vi "Schema.vi"(8 "error in (no error)":errorcluster, 11 "SQLite Connection In":refnum<class "Connection.lvclass">) -> (0 "error out":errorcluster, 1 "Table Names":string[](array[string]), 2 "Schema":T1, 3 "SQLite Connection Out":refnum<class "Connection.lvclass">)   [LabVIEW 2024, in "DBMigrations.lvlib"]
doc: "Get database schema: table names, column names, and column properties"
uses:
  DBMigrations.lvlib
  <vilib>/drjdpowell/SQLite Library/SQL Connection/Connection.lvclass
  Schema.ctl
  <vilib>/drjdpowell/SQLite Library/SQL Connection/Execute SQL (1D String).vi
  <vilib>/drjdpowell/SQLite Library/SQL Connection/Execute SQL.vi
  <vilib>/drjdpowell/SQLite Library/SQLite.lvlib
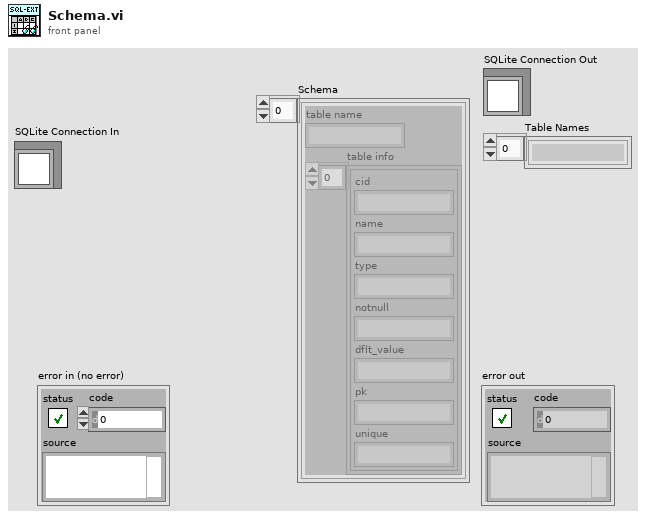
[diagram p1: front panel]
types:
  T1 = typedef "DBMigrations.lvlib/Schema.ctl" = cluster{"table name":string, "table info":cluster{"cid":string, "name":string, "type":string, "notnull":string, "dflt_value":string, "pk":string, "unique":string}[]}[]
  T2 = cluster{"table name":string, "table info":cluster{"cid":string, "name":string, "type":string, "notnull":string, "dflt_value":string, "pk":string, "unique":string}[]}
  T3 = cluster{"cid":string, "name":string, "type":string, "notnull":string, "dflt_value":string, "pk":string, "unique":string}
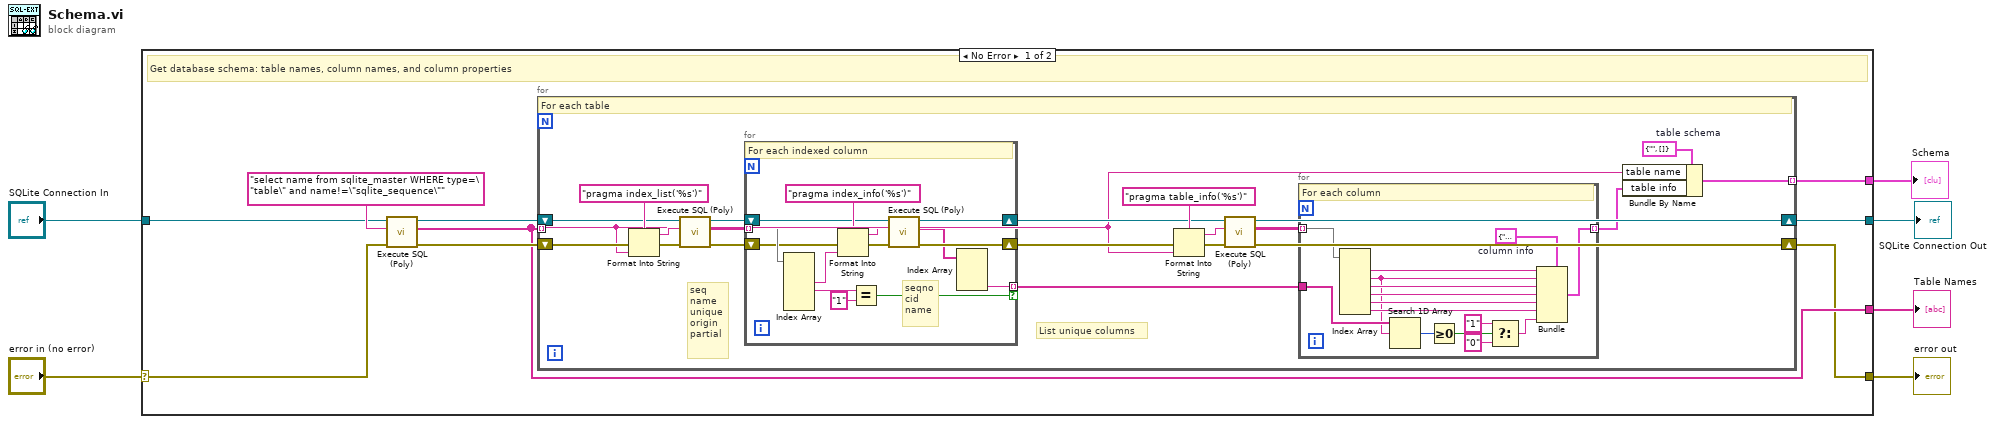
[diagram p0: block diagram]
diagram:
  n1 = case shown="No Error" "error in (no error)" {
    selector: "error in (no error)" -> [w15 w67]
    tunnel: [w9 w67] -> w5
    tunnel: "SQLite Connection In" -> [w8 w66]
    tunnel: [w11 _] -> w1
    tunnel: [w10 _] -> w4
    tunnel: [w7 w66] -> w2
    frame No Error {
      # "Get database schema: table names, column names, and column properties"
      n2 = call-poly <vilib>:"Execute SQL (Poly).vi"("error in (no error)"=w15, "SQL"="select name from sqlite_master WHERE type=\"table\" and name!=\"sqlite_sequence\"", "SQLite Connection in"=w8) -> ("error out"=w12:errorcluster, "Result Set"=w10:string[], "SQLite Connection"=w13:refnum<class "Connection.lvclass">)  [unwired: 5 in, 1 out]
      n3 = for {
        shift-right: [w36] -> w7
        shift-left: w13 -> [w21]
        shift-right: [w35] -> w9
        shift-left: w12 -> [w20]
        tunnel: w10 -> [w16] mode=indexing
        tunnel: [w29] -> w11 mode=indexing
        w28 = T2 {"table name"="", "table info"=[]}  # table schema
        # "List unique columns"
        # "seq\nname\nunique\norigin\npartial"
        # "For each table"
        n4 = Format Into String(format string="pragma index_list('%s')", error in=w20, w16) -> (resulting string=w23:string, error out=w24:errorcluster)  [unwired: 1 in]
        n5 = call-poly <vilib>:"Execute SQL (Poly).vi"("error in (no error)"=w24, "SQL"=w23, "SQLite Connection in"=w21) -> ("error out"=w27:errorcluster, "Result Set"=w25:string[][], "SQLite Connection"=w26:refnum<class "Connection.lvclass">)  [unwired: 5 in, 1 out]
        n6 = for {
          tunnel: w25 -> [w50] mode=indexing
          shift-right: [w44] -> w19
          shift-left: w26 -> [w45]
          shift-right: [w43] -> w18
          shift-left: w27 -> [w42]
          tunnel: [w40] -> w17 mode=indexing if=w37
          # "seqno\ncid\nname"
          # "For each indexed column"
          n7 = Index Array(array=w50) -> (element #2=w46:string, element #3=w39:string)  [unwired: 5 in, 3 out]
          n8 = Format Into String(format string="pragma index_info('%s')", error in=w42, w46) -> (resulting string=w49:string, error out=w48:errorcluster)  [unwired: 1 in]
          n9 = Equal?(x=w39, y="1") -> (x = y?=w37:bool)
          n10 = call-poly <vilib>:"Execute SQL (Poly).vi"("error in (no error)"=w48, "SQL"=w49, "SQLite Connection in"=w45) -> ("error out"=w43:errorcluster, "Result Set"=w41:string[], "SQLite Connection"=w44:refnum<class "Connection.lvclass">)  [unwired: 5 in, 1 out]
          n11 = Index Array(array=w41) -> (element #3=w40:string)  [unwired: 3 in, 2 out]
        }
        n12 = Format Into String(format string="pragma table_info('%s')", error in=w18, w16) -> (resulting string=w31:string, error out=w32:errorcluster)  [unwired: 1 in]
        n13 = call-poly <vilib>:"Execute SQL (Poly).vi"("error in (no error)"=w32, "SQL"=w31, "SQLite Connection in"=w19) -> ("error out"=w35:errorcluster, "Result Set"=w34:string[][], "SQLite Connection"=w36:refnum<class "Connection.lvclass">)  [unwired: 5 in, 1 out]
        n14 = for {
          tunnel: w34 -> [w65] mode=indexing
          tunnel: [w64] -> w33 mode=indexing
          tunnel: w17 -> [w57]
          w58 = T3 {"cid"="", "name"="", "type"="", "notnull"="", "dflt_value"="", "pk"="", "unique"=""}  # column info
          # "For each column"
          n15 = Index Array(array=w65) -> (element #1=w63:string, element #2=w56:string, element #3=w62:string, element #4=w61:string, element #5=w60:string, element #6=w59:string)  [unwired: 6 in]
          n16 = Search 1D Array(1D array=w57, element=w56) -> (index of element=w55:i32)  [unwired: 1 in]
          n17 = Greater Or Equal To 0?(x=w55) -> (x >= 0?=w54:bool)
          n18 = Select(t="1", s=w54, f="0") -> (s? t:f=w51:string)
          n19 = Bundle(cluster=w58, "cid"=w63, "name"=w56, "type"=w62, "notnull"=w61, "dflt_value"=w60, "pk"=w59, "unique"=w51) -> (w64:T3)
        }
        n20 = Bundle By Name(cluster=w28, "table name"=w16, "table info"=w33) -> (w29:T2)
      }
    }
    frame Error {
    }
  }
  "error out" <- w5
  "Table Names" <- w4
  "SQLite Connection Out" <- w2
  "Schema" <- w1
